vi "Launch Fault Insertion IO.vi"(11 "Fault-Injection Bus":refnum<class "Fault-Injection Bus.lvclass">) -> ()   [LabVIEW 2021]
uses:
  <vilib>/TSA/Omni-Bus/Fault-Injection Bus/Fault-Injection Bus.lvclass
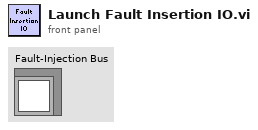
[diagram p1: front panel]
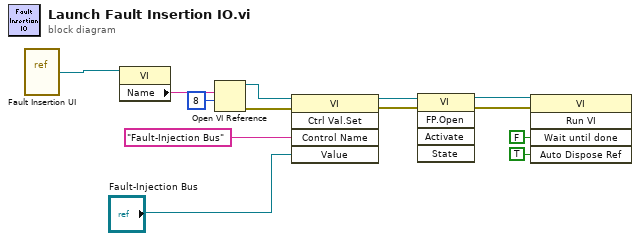
[diagram p0: block diagram]
diagram:
  n1 = vi-ref "Fault Insertion UI.vi"() -> (w1:refnum<vi>)
  n2 = property class="VI"(reference=w1) -> ("Name"=w3:string)  [unwired: 1 in, 2 out]
  n3 = Open VI Reference(vi path=w3, options=8) -> (vi reference=w4:refnum<vi>, error out=w5:errorcluster)  [unwired: 4 in]
  n4 = invoke class="VI" method="Ctrl Val.Set"(reference=w4, error in=w5, "Control Name"="Fault-Injection Bus", "Value"="Fault-Injection Bus") -> (reference out=w10:refnum<vi>, error out=w11:errorcluster)  [unwired: 1 in, 3 out]
  n5 = invoke class="VI" method="FP.Open"(reference=w10, error in=w11) -> (reference out=w12:refnum<vi>, error out=w13:errorcluster)  [unwired: 3 in, 3 out]
  n6 = invoke class="VI" method="Run VI"(reference=w12, error in=w13, "Wait until done"=FALSE ("Wait Until Done"), "Auto Dispose Ref"=TRUE ("Auto Dispose Reference")) -> ()  [unwired: 1 in, 5 out]
